vi "Write Device Metadata.vi"(0 "File Path":path, 11 "Error In":errorcluster) -> (4 "File Path (Dup)":path, 15 "Write Errror":errorcluster)   [LabVIEW 2016]
uses:
  Device Metadata Types/Device Metadata.ctl
  Device Metadata Types/AOTF Metadata.ctl
  Device Metadata Types/Basic Device Info.ctl
  Device Metadata Types/AOTF Channel Metadata.ctl
  Device Metadata Types/Camera Metadata.ctl
  Device Library/Cameras/Camera Controls/Generic Camera ROI.ctl
  Device Metadata Types/Lasers Metadata.ctl
  Device Metadata Types/Shutter Metadata.ctl
  Device Metadata Types/Stages Metadata.ctl
  Hardware Configuration/Hardware Configuration Controls/Device Type.ctl
  Device Library/AOTFs/AOTF Controls/AOTF Actions.ctl
  Device Library/Cameras/Camera Controls/Generic Camera Actions.ctl
  Device Library/Lasers/Laser Controls/Laser Actions.ctl
  Device Library/Shutters/Shutter Controls/Shutter Actions.ctl
  Device Library/Stages/Stages Controls/Stage Actions.ctl
  shell32.dll
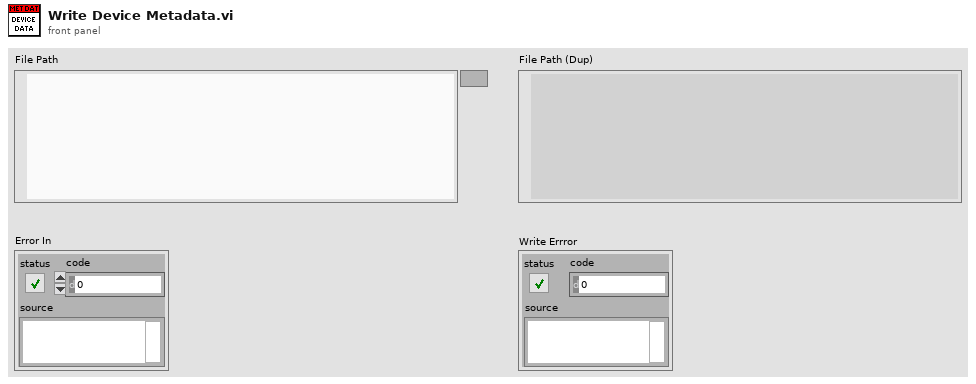
[diagram p1: front panel]
types:
  T1 = typedef "Device Metadata.ctl" = cluster{"AOTF":T2[], "Cameras":T5[], "Lasers":T7[], "Shutters":T8[], "Stages":T9[]}
  T2 = typedef "AOTF Metadata.ctl" = cluster{"Basic_Info":T3, "Beam_Blank":bool, "Channel_Info":T4[]}
  T3 = typedef "Basic Device Info.ctl" = cluster{"Device_Type":string, "Function":string, "Company":string}
  T4 = typedef "AOTF Channel Metadata.ctl" = cluster{"Wavelength_nm":string, "Power_Percent":dbl, "Line_On_Off":bool}
  T5 = typedef "Camera Metadata.ctl" = cluster{"Basic_Info":T3, "Exposure_Time_sec":dbl, "Running":bool, "General_Camera_ROI":T6}
  T6 = typedef "Generic Camera ROI.ctl" = cluster{"H_Offset":u16, "V_Offset":u16, "H_Width":u16, "V_Width":u16}
  T7 = typedef "Lasers Metadata.ctl" = cluster{"Basic_Info":T3, "Enabled_Interlock":bool, "Light_Emission":bool, "Power_mW":dbl, "Laser_Status":string}
  T8 = typedef "Shutter Metadata.ctl" = cluster{"Basic_Info":T3, "Open":bool}
  T9 = typedef "Stages Metadata.ctl" = cluster{"Basic_Info":T3, "Positions":dbl[]}
  T10 = typedef "Device Type.ctl" = enum16{"AOTF", "Camera", "Deformable Mirror", "Laser", "Shutter", "Stage", "Waveform", "FPGA", "Email", "Filter Wheel"}
  T11 = typedef "Generic Camera Actions.ctl" = enum16{"Status", "Live Preview", "Capture", "Abort", "Set Exposure Time (s)", "Get Exposure Time (s)", "Record Settings", "Binning", "Set ROI", "Get ROI", "Defect Correction On?", "Cooler On?", "Fan On?", "Quit"}
  T12 = typedef "Laser Actions.ctl" = enum16{"Error Check", "Set On/Off", "Set Power", "Set Parameter", "Get Power", "Get Status", "Get Parameter", "Quit"}
  T13 = typedef "Shutter Actions.ctl" = enum16{"Open", "Close", "Toggle", "Status", "Quit"}
  T14 = typedef "Stage Actions.ctl" = enum16{"Get Position", "MVR", "MOVE", "HALT", "ONTARGET", "ERROR", "REFERENCE", "INIT", "VELOCITY", "STATUS", "EXIT", "HOME", "ZEROPOS", "NANOPOS", "ANALOG", "QUIT"}
  T15 = typedef "AOTF Actions.ctl" = enum16{"Error Check", "Blank", "Line On/Off", "Set Power", "Status", "Quit"}
  T16 = typedef "Laser Status.ctl" = enum16{"Warmup", "Ready", "Emission", "Tuning", "Error"}
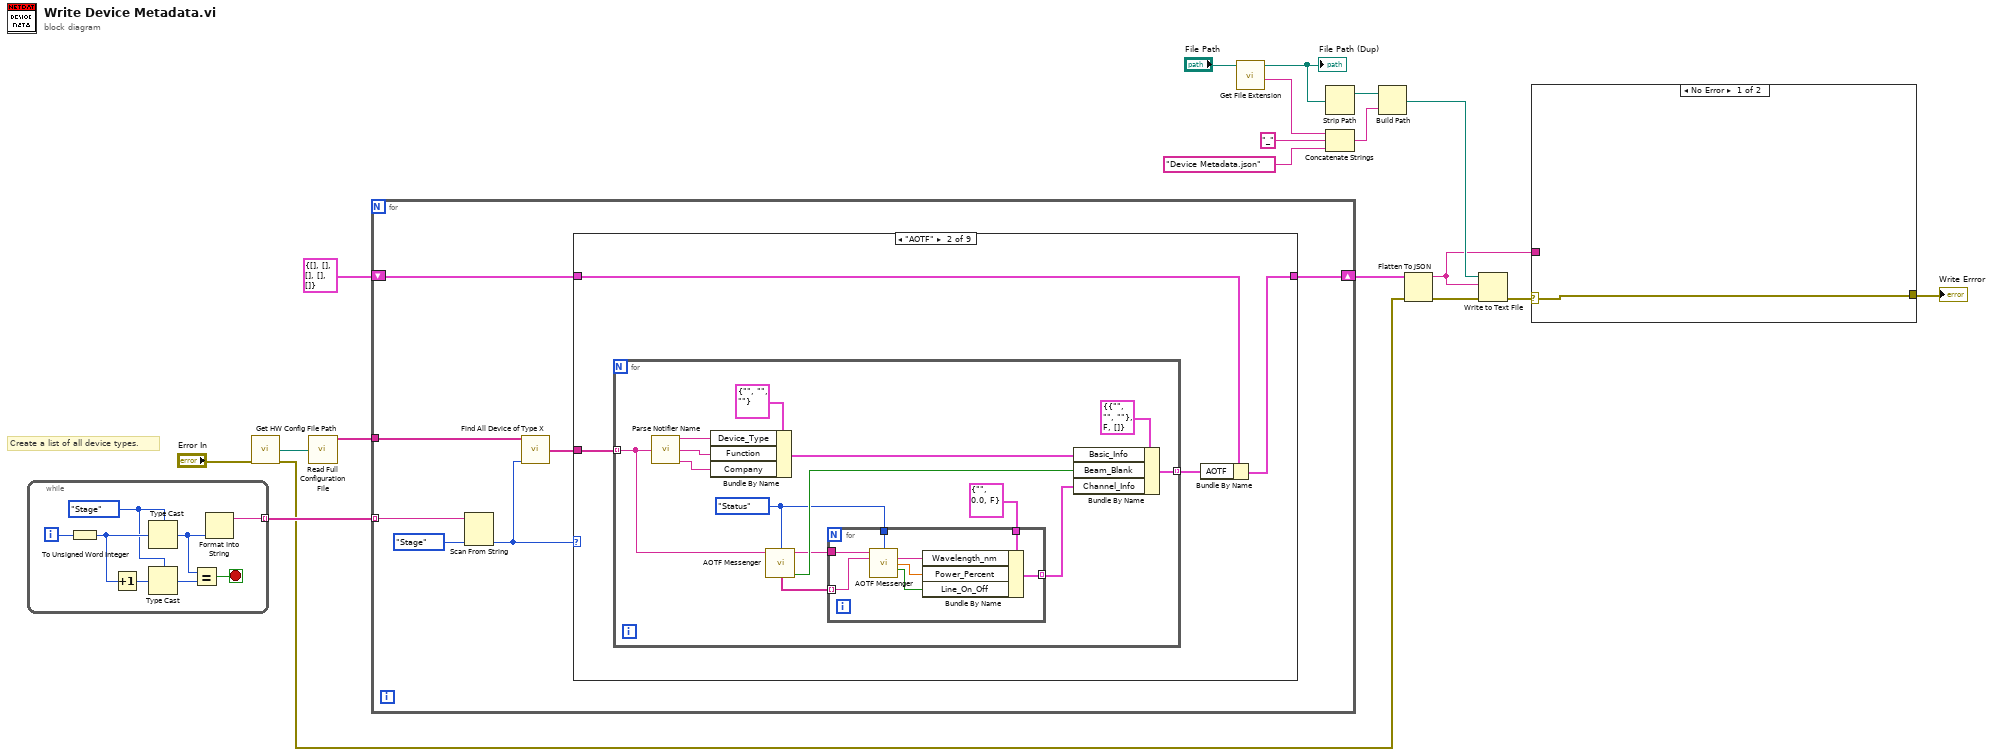
[diagram p0: block diagram]
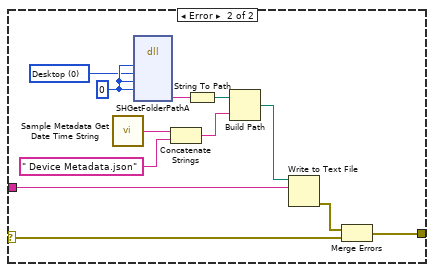
[diagram p2: hidden frame]
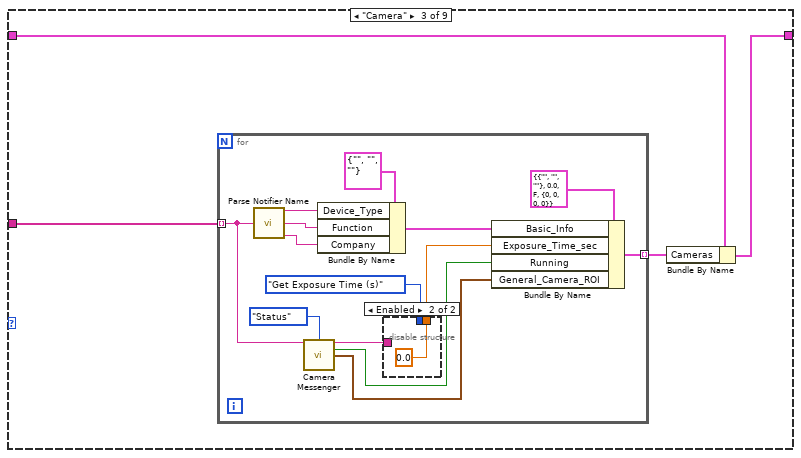
[diagram p4: hidden frame]
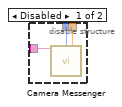
[diagram p5: hidden frame]
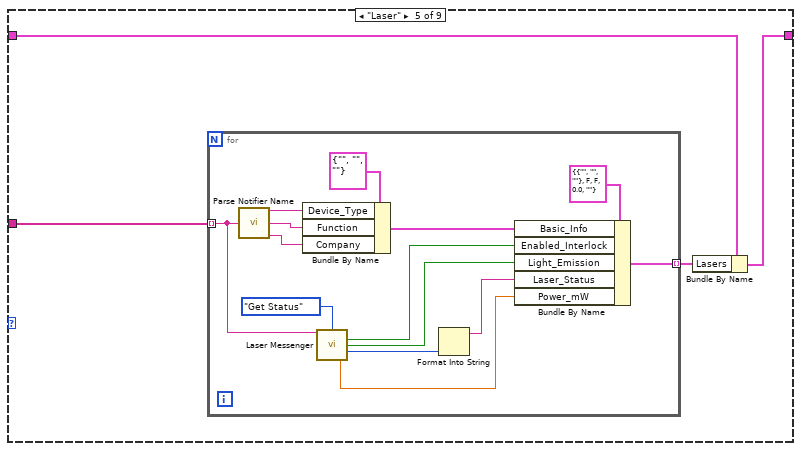
[diagram p7: hidden frame]
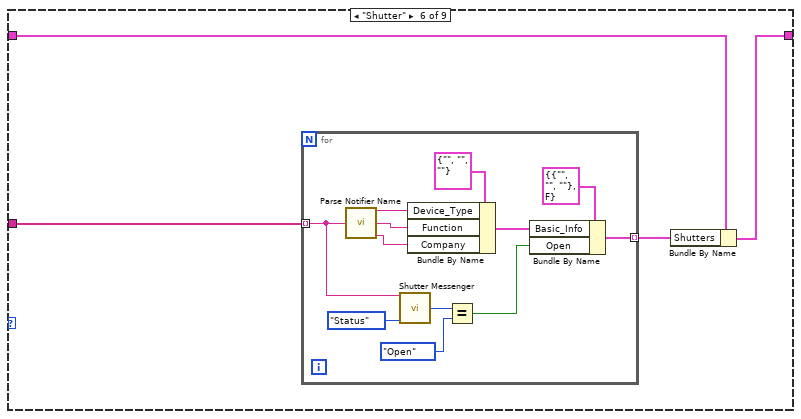
[diagram p8: hidden frame]
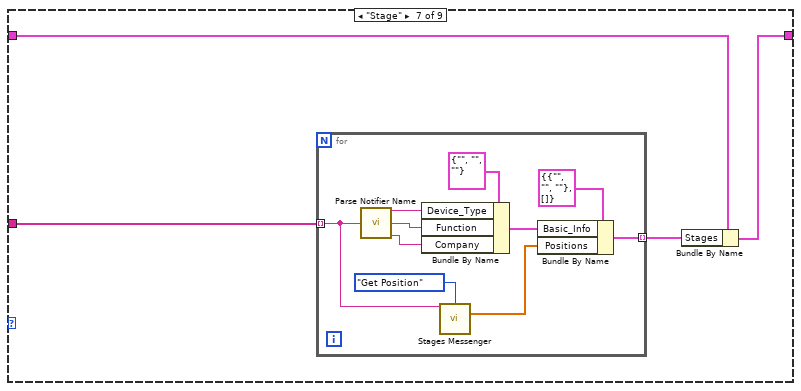
[diagram p9: hidden frame]
diagram:
  # "Create a list of all device types."
  n1 = while {
    tunnel: [w20] -> w19 mode=indexing
    i -> [w23]
    stop <- w22 stop-if-true
    w24 = Device_Type."Stage" ("Device Type")
    n2 = To Unsigned Word Integer(number=w23) -> (unsigned 16bit integer=w25:u16)
    n3 = Increment(x=w25) -> (x+1=w26:u16)
    n4 = Type Cast(type=w24, x=w25) -> (*(type *) &x=w21:T10)
    n5 = Type Cast(type=w24, x=w26) -> (*(type *) &x=w27:T10)
    n6 = Equal?(x=w21, y=w27) -> (x = y?=w22:bool)
    n7 = Format Into String(w21) -> (resulting string=w20:string)  [unwired: 3 in, 1 out]
  }
  n8 = call "Get HW Config File Path.vi"("Error"="Error In") -> ("File Path"=w18:path, "Error"=w4:errorcluster)  [unwired: 13 in]
  n9 = call "Read Full Configuration File.vi"("Config File Path"=w18) -> ("Unique Notifier Names"=w17:string[])  [unwired: 11 in, 3 out]
  n10 = for {
    tunnel: w19 -> [w34] mode=indexing
    tunnel: w17 -> [w31]
    shift-right: [w28] -> w15
    shift-left: T1 {"AOTF"=[], "Cameras"=[], "Lasers"=[], "Shutters"=[], "Stages"=[]} ("Device Metadata") -> [w29]
    n11 = Scan From String(input string=w34, default 1=Device_Type."Stage" ("Device Type")) -> (output 1=w32:T10)  [unwired: 3 in, 3 out]
    n12 = call "Find All Device of Type X.vi"("Unique Notifier Names"=w31, "Device Type"=w32) -> ("Running Devices"=w30:string[])  [unwired: 12 in, 1 out]
    n13 = case shown="\"AOTF\"" w32 {
      tunnel: w30 -> [_ w39 w65 _ w88 w106 w122 _ _]
      tunnel: w29 -> [w35 w38 w64 w84 w87 w105 w121 w133 w134]
      tunnel: [w35 w36 w62 w84 w85 w103 w119 w133 w134] -> w28
      frame Default {
      }
      frame "AOTF" {
        n14 = for {
          tunnel: w39 -> [w53] mode=indexing
          tunnel: [w40] -> w37 mode=indexing
          w41 = AOTF_Actions."Status" ("AOTF Action")
          n15 = call "Parse Notifier Name.vi"("Notifier Name"=w53) -> ("Device Type"=w50:string, "Function"=w51:string, "Company"=w52:string)  [unwired: 12 in]
          n16 = Bundle By Name(cluster=T3 {"Device_Type"="", "Function"="", "Company"=""} ("Basic Info"), "Device_Type"=w50, "Function"=w51, "Company"=w52) -> (w47:T3)
          n17 = call "AOTF Messenger.vi"("AOTF Notifier Name"=w53, "AOTF Action"=w41) -> ("AOTF Notifier Name (Dup)"=w44:string, "Wavelengths (nm)"=w45:string[], "Beam Blank Out"=w46:bool)  [unwired: 8 in, 3 out]
          n18 = for {
            tunnel: w45 -> [w59] mode=indexing
            tunnel: w44 -> [w60]
            tunnel: T4 {"Wavelength_nm"="", "Power_Percent"=0.0, "Line_On_Off"=FALSE} ("Channel Data") -> [w61]
            tunnel: [w55] -> w42 mode=indexing
            tunnel: w41 -> [w54]
            n19 = call "AOTF Messenger.vi"("AOTF Notifier Name"=w60, "AOTF Action"=w54, "Wavelength (nm)"=w59) -> ("Wavelength (nm) Out"=w58:string, "Power (%) Out"=w56:dbl, "Line On/Off Out"=w57:bool)  [unwired: 7 in, 3 out]
            n20 = Bundle By Name(cluster=w61, "Wavelength_nm"=w58, "Power_Percent"=w56, "Line_On_Off"=w57) -> (w55:T4)
          }
          n21 = Bundle By Name(cluster=T2 {"Basic_Info"={"Device_Type"="", "Function"="", "Company"=""}, "Beam_Blank"=FALSE, "Channel_Info"=[]} ("AOTF Metadata"), "Basic_Info"=w47, "Beam_Blank"=w46, "Channel_Info"=w42) -> (w40:T2)
        }
        n22 = Bundle By Name(cluster=w38, "AOTF"=w37) -> (w36:T1)
      }
      frame "Camera" {
        n23 = for {
          tunnel: w65 -> [w74] mode=indexing
          tunnel: [w66] -> w63 mode=indexing
          n24 = call "Parse Notifier Name.vi"("Notifier Name"=w74) -> ("Device Type"=w77:string, "Function"=w78:string, "Company"=w79:string)  [unwired: 12 in]
          n25 = call "Camera Messenger.vi"("Notifier Name"=w74, "General Camera Actions"=Generic_Camera_Actions."Status") -> ("Notifier Name Dup"=w72:string, "Running?"=w67:bool, "Camera ROI"=w68:T6)  [unwired: 8 in, 3 out]
          n26 = Bundle By Name(cluster=T3 {"Device_Type"="", "Function"="", "Company"=""} ("Basic Info"), "Device_Type"=w77, "Function"=w78, "Company"=w79) -> (w70:T3)
          n27 = disable-structure shown="Enabled" {
            disable-tunnel: Generic_Camera_Actions."Get Exposure Time (s)" ("General Camera Actions") -> [w82 _]
            disable-tunnel: w72 -> [w81 _]
            disable-tunnel: [w80 0.0] -> w69
            frame Disabled {
              n28 = call "Camera Messenger.vi"("Notifier Name"=w81, "General Camera Actions"=w82) -> ("Current Exposure Time (s)"=w80:dbl)  [unwired: 8 in, 5 out]
            }
            frame Enabled {
            }
          }
          n29 = Bundle By Name(cluster=T5 {"Basic_Info"={"Device_Type"="", "Function"="", "Company"=""}, "Exposure_Time_sec"=0.0, "Running"=FALSE, "General_Camera_ROI"={"H_Offset"=0, "V_Offset"=0, "H_Width"=0, "V_Width"=0}} ("Camera Metadata"), "Basic_Info"=w70, "Exposure_Time_sec"=w69, "Running"=w67, "General_Camera_ROI"=w68) -> (w66:T5)
        }
        n30 = Bundle By Name(cluster=w64, "Cameras"=w63) -> (w62:T1)
      }
      frame "Deformable Mirror" {
      }
      frame "Laser" {
        n31 = for {
          tunnel: w88 -> [w98] mode=indexing
          tunnel: [w94] -> w86 mode=indexing
          n32 = call "Parse Notifier Name.vi"("Notifier Name"=w98) -> ("Device Type"=w100:string, "Function"=w101:string, "Company"=w102:string)  [unwired: 12 in]
          n33 = Bundle By Name(cluster=T3 {"Device_Type"="", "Function"="", "Company"=""} ("Basic Info"), "Device_Type"=w100, "Function"=w101, "Company"=w102) -> (w95:T3)
          n34 = call "Laser Messenger.vi"("Notifier Name"=w98, "Action"=Laser_Actions."Get Status") -> ("Enabled (Interlock)?"=w93:bool, "Light Emission?"=w92:bool, "Laser Status"=w90:T16, "Power (mW)"=w91:dbl)  [unwired: 8 in, 2 out]
          n35 = Format Into String(w90) -> (resulting string=w89:string)  [unwired: 3 in, 1 out]
          n36 = Bundle By Name(cluster=T7 {"Basic_Info"={"Device_Type"="", "Function"="", "Company"=""}, "Enabled_Interlock"=FALSE, "Light_Emission"=FALSE, "Power_mW"=0.0, "Laser_Status"=""} ("Laser Metadata"), "Basic_Info"=w95, "Enabled_Interlock"=w93, "Light_Emission"=w92, "Laser_Status"=w89, "Power_mW"=w91) -> (w94:T7)
        }
        n37 = Bundle By Name(cluster=w87, "Lasers"=w86) -> (w85:T1)
      }
      frame "Shutter" {
        n38 = for {
          tunnel: w106 -> [w112] mode=indexing
          tunnel: [w107] -> w104 mode=indexing
          n39 = call "Parse Notifier Name.vi"("Notifier Name"=w112) -> ("Device Type"=w117:string, "Function"=w116:string, "Company"=w115:string)  [unwired: 12 in]
          n40 = call "Shutter Messenger.vi"("Notifier Name"=w112, "Action"=Shutter_Actions."Status") -> ("Shutter Status"=w110:T13)  [unwired: 12 in, 1 out]
          n41 = Bundle By Name(cluster=T3 {"Device_Type"="", "Function"="", "Company"=""} ("Basic Info"), "Device_Type"=w117, "Function"=w116, "Company"=w115) -> (w113:T3)
          n42 = Equal?(x=w110, y=Shutter_Actions."Open") -> (x = y?=w108:bool)
          n43 = Bundle By Name(cluster=T8 {"Basic_Info"={"Device_Type"="", "Function"="", "Company"=""}, "Open"=FALSE} ("Shutter Metadata"), "Basic_Info"=w113, "Open"=w108) -> (w107:T8)
        }
        n44 = Bundle By Name(cluster=w105, "Shutters"=w104) -> (w103:T1)
      }
      frame "Stage" {
        n45 = for {
          tunnel: w122 -> [w132] mode=indexing
          tunnel: [w123] -> w120 mode=indexing
          n46 = call "Parse Notifier Name.vi"("Notifier Name"=w132) -> ("Device Type"=w129:string, "Function"=w127:string, "Company"=w128:string)  [unwired: 12 in]
          n47 = Bundle By Name(cluster=T3 {"Device_Type"="", "Function"="", "Company"=""} ("Basic Info"), "Device_Type"=w129, "Function"=w127, "Company"=w128) -> (w125:T3)
          n48 = call "Stages Messenger.vi"("Stage Notifier Name"=w132, "Actions"=Stage_Actions."Get Position") -> ("Positions"=w124:dbl[])  [unwired: 10 in, 3 out]
          n49 = Bundle By Name(cluster=T9 {"Basic_Info"={"Device_Type"="", "Function"="", "Company"=""}, "Positions"=[]} ("Stage Metadata"), "Basic_Info"=w125, "Positions"=w124) -> (w123:T9)
        }
        n50 = Bundle By Name(cluster=w121, "Stages"=w120) -> (w119:T1)
      }
      frame "Waveform" {
      }
      frame "Email" {
      }
    }
  }
  n51 = call <vilib>:"Get File Extension.vi"("file"="File Path") -> ("filename without extension"=w8:string, "dup file"=w9:path)  [unwired: 6 in, 3 out]
  "File Path (Dup)" <- w9
  n52 = Strip Path(path=w9) -> (stripped path=w13:path)  [unwired: 1 out]
  n53 = Concatenate Strings(w8, "_" ("string"), "Device Metadata.json" ("name or relative path")) -> (w11:string)
  n54 = Build Path(base path=w13, name or relative path=w11) -> (appended path=w6:path)
  n55 = Flatten To JSON(anything=w15, error in (no error)=w4) -> (JSON string=w2:string, 11:w14:errorcluster)  [unwired: 1 in]
  n56 = Write to Text File(file (use dialog)=w6, text=w2, error in=w14) -> (error out=w3:errorcluster)  [unwired: 1 in, 2 out]
  n57 = case shown="No Error" w3 {
    selector: w3 -> [w135 w137]
    tunnel: w2 -> [_ w147]
    tunnel: [w135 w136] -> w1
    frame No Error {
    }
    frame Error {
      w143 = 0 items=["Desktop"=0, "Personal Documents"=5, "AppData"=26, "Local AppData"=28, "Common AppData"=35, "Program Files"=38, "Program Files Common"=43, "Common Documents"=46] ("Requested Path")
      w144 = 0 ("HWND")
      n58 = call "Sample Metadata Get Date Time String.vi"() -> ("Date Time String"=w140:string)  [unwired: 15 in]
      n59 = dll-call lib="shell32.dll" fn="SHGetFolderPathA"("HWND"=w144, "nFolder"=w143, "hToken"=w144, "dwFlags"=w144) -> ("pszPath"=w145:string)  [unwired: 9 in, 2 out]
      n60 = Concatenate Strings(w140, " Device Metadata.json" ("string")) -> (w139:string)
      n61 = String To Path(string=w145) -> (path=w146:path)
      n62 = Build Path(base path=w146, name or relative path=w139) -> (appended path=w142:path)
      n63 = Write to Text File(file (use dialog)=w142, text=w147) -> (error out=w138:errorcluster)  [unwired: 2 in, 2 out]
      n64 = Merge Errors(w138, w137) -> (w136:errorcluster)
    }
  }
  "Write Errror" <- w1
